vi "Write DAQ FIFO.vi"(6 "FIFO Timestamps":T2, 8 "error in (no error)":errorcluster, 9 "Timeout (ms)":i32, 10 "Data In":T1[](array[typedef]), 11 "CIFFIFO in":refnum<class "CIF_CIPC_Fifo_DAQ.lvclass">) -> (0 "error out":errorcluster, 1 "timed out?":bool, 2 "Data Out":T1[](array[typedef]), 3 "CIFFIFO out":refnum<class "CIF_CIPC_Fifo_DAQ.lvclass">)   [LabVIEW 2021, in "CIF_CIPC_Fifo_DAQ.lvclass"]
uses:
  CIF_CIPC_Fifo_DAQ.lvclass
  <vilib>/CIF Foundation/CIF Channels Core/ChannelCommon/typedef/TimeStamps.ctl
  D:/dev/Packages/CIF_Channels_CIPC/src/CIPC_Channels/CIF_CIPC_Chan/CIF_CIPC_Chn.lvclass
  C:/Program Files/National Instruments/LabVIEW 2021/vi.lib/CIF Foundation/CIF Channels Core/CIFChannels/CIFChannels.lvclass
  <vilib>/CIF Foundation/CIF Channels Core/ChannelCommon/typedef/Datatype Waveform.ctl
  <vilib>/CIF Foundation/CIF Channels Core/CIFChannels/CIFChannels.lvclass/CIFChannels.ctl
  CIF_CIPC_Chan/CIF_CIPC_Chn.lvclass/CIF_CIPC_Chn.ctl
  <vilib>/CIF Foundation/CIF Utilities/Statistics/I64/Stats_I64_CIF_U.lvclass/Stats_I64_CIF_U.ctl
  CIF_CIPC_Chan/Accessors/Read Buffer Configuration.vi
  CIF_CIPC_Chan/SubVIs/Check Writer Backpressure.vi/7796537b-0e69-421b-96bb-30a861203fb6.vi
  <vilib>/CIF Foundation/CIF Channels Core/CIFChannels/Accessors/Read FIFO Backpressure.vi
  <vilib>/CIF Foundation/CIF Channels Core/CIFChannels/Utilities/Update Channel Benchmark.vi
  SubVIs/Core Write DAQ FIFO.vi/1bad10da-a98b-49ee-b03a-18b497e396df.vi
  SubVIs/Core Write DAQ FIFO.vi/70f860b1-5d4a-43dc-b0c2-c9446e8447f7.vi
  CIF_CIPC_Chan/Accessors/Read CIPC Channel.vi
  SubVIs/Write One DAQ Waveform.vi
  CIF_CIPC_Chan/SubVIs/Write FIFO Header to CIPC.vi/2516c5c4-bcd6-4eab-a054-fa3d4f1376bc.vi
  CIF_CIPC_Chan/SubVIs/Check Writer Backpressure.vi/7796537b-0e69-421b-96bb-30a861203fb6.vi/a816fde8-6378-45f6-992d-c1f6c5777b8d.vi
  <vilib>/CIF Foundation/CIF CIPC/SubVIs/Get Element Write Position.vi
  <vilib>/CIF Foundation/CIF CIPC/Utilities/Get Size.vi
  <vilib>/CIF Foundation/CIF Utilities/Statistics/I64/X1 minus X0.vi
  <vilib>/CIF Foundation/CIF Utilities/Time/System Time/Get System Time.vi
  SubVIs/Write One DAQ Waveform.vi/296b4b7f-f24e-461b-ac09-61c48c94f223.vi
  SubVIs/Write One DAQ Waveform.vi/489ce88f-d13b-4e3d-8a44-beac6fbb575f.vi
  <vilib>/CIF Foundation/CIF CIPC/SubVIs/Check Error.vi
  <vilib>/CIF Foundation/CIF CIPC/SubVIs/Notify Of New Write.vi
  <vilib>/CIF Foundation/CIF CIPC/SubVIs/Get dll Path.vi
  <vilib>/CIF Foundation/CIF CIPC/SubVIs/Wait For N Elements Available.vi
  <vilib>/CIF Foundation/CIF CIPC/SubVIs/Get Element Read Position.vi
  <vilib>/CIF Foundation/CIF CIPC/SubVIs/Set Element Read Position.vi
  <vilib>/CIF Foundation/CIF Utilities/Statistics/I64/X1 minus X0.vi/dfabcf33-0dbc-4041-80a5-3dc0c86d2989.vi
  <vilib>/CIF Foundation/CIF Utilities/Statistics/I64/X1 minus X0.vi/dfabcf33-0dbc-4041-80a5-3dc0c86d2989.vi/9eb60a9a-770f-4d2d-8b3f-8465c267ecc9.vi
  CIF_CIPC_Chan/CIF_CIPC_Chn.lvclass
  <vilib>/CIF Foundation/CIF CIPC/SubVIs/Check Error Core.vi
  <vilib>/CIF Foundation/CIF CIPC/SubVIs/Get Element Info Variant.vi
  <vilib>/CIF Foundation/CIF CIPC/SubVIs/Check Backpressure FIFO Space.vi
  <vilib>/CIF Foundation/CIF Channels Core/CIFChannels/Utilities/Create Flattened FIFO Header.vi
  <vilib>/CIF Foundation/CIF Channels Core/ChannelCommon/ChannelCommon.lvlib
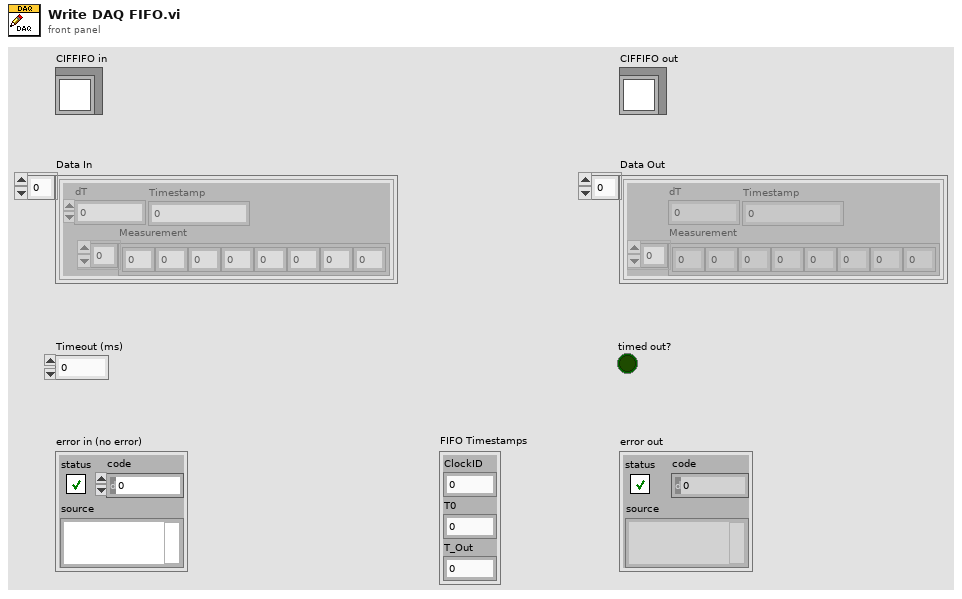
[diagram p1: front panel]
types:
  T1 = typedef "ChannelCommon.lvlib/Datatype Waveform.ctl" = cluster{"Measurement":dbl[], "dT":dbl, "Timestamp":i64}
  T2 = typedef "ChannelCommon.lvlib/TimeStamps.ctl" = cluster{"ClockID":u8, "T0":i64, "T_Out":i64}
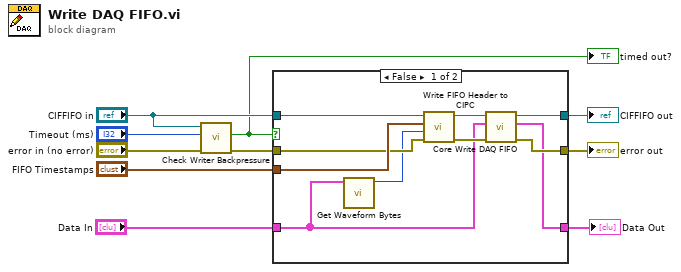
[diagram p0: block diagram]
diagram:
  n1 = call "Check Writer Backpressure.vi"("error in (no error)"="error in (no error)", "Timeout (ms)"="Timeout (ms)", "CIF_CIPC_Chn in"="CIFFIFO in") -> ("error out"=w10:errorcluster, "timed out?"=w5:bool)  [unwired: 7 in]
  "timed out?" <- w5
  n2 = case shown="False" w5 {
    tunnel: [w20 w23] -> w3
    tunnel: [w19 w22] -> w4
    tunnel: "FIFO Timestamps" -> [w18 _]
    tunnel: "Data In" -> [w11 w21]
    tunnel: "CIFFIFO in" -> [w15 w22]
    tunnel: w10 -> [w14 w23]
    tunnel: [w13 w21] -> w1
    frame False {
      n3 = call <vilib>:"Get Waveform Bytes.vi"("Waveforms"=w11) -> ("Bytes"=w12:i32)  [unwired: 10 in]
      n4 = call "Write FIFO Header to CIPC.vi"("error in (no error)"=w14, "Payload Length (bytes)"=w12, "FIFO Timestamps"=w18, "CIF_CIPC_Chn in"=w15) -> ("error out"=w16:errorcluster, "CIF_CIPC_Chn out"=w17:refnum<class "CIF_CIPC_Fifo_DAQ.lvclass">)  [unwired: 6 in]
      n5 = call "Core Write DAQ FIFO.vi"("error in (no error)"=w16, "Data In"=w11, "CIFFIFO in"=w17) -> ("error out"=w20:errorcluster, "Data Out"=w13:T1[], "CIFFIFO out"=w19:refnum<class "CIF_CIPC_Fifo_DAQ.lvclass">)  [unwired: 6 in]
    }
    frame True {
    }
  }
  "error out" <- w3
  "CIFFIFO out" <- w4
  "Data Out" <- w1
